vi "DAT Example.vi"() -> ()   [LabVIEW 2019]
uses:
  LV-Data/Typedefs/File Type--enum.ctl
  LV-Data/Typedefs/Dictionary--cluster.ctl
  LV-Data/LV-Data.lvclass
panel:
  out "data rows saved":i32
  in  "stop":bool
  in  "number4":dbl=7.0
  in  "number3":dbl=5.0
  in  "number2":dbl=3.0
  in  "number1":dbl
  in  "wavenames (.Vx, etc)":string[](array[string])=["time", "temp", "Bfield", "X0", "Y0", "X1", "Y1", "X2", "Y2", "X3", "Y3", "X4", "Y4", "X5", "Y5"]
  out "plot2":cluster{"X":dbl[], "Y":dbl[]}[](graph)
  out "plot1":cluster{"X":dbl[], "Y":dbl[]}[](graph)
  out "plot0":cluster{"X":dbl[], "Y":dbl[]}[](graph)
  in  "Notes":string="date and time are AUTOMATICALLY saved!\nwrite your experiment notes here"
  in  "path":path=path "C:/"
  in  "filename":string="datatest"
  # "- set path to folder\n- set base filename\n   (up to 999,999 files with same base name \n    an be written in one folder)\n- type some comments"
  # "you usually display your data as a XY\ngraphs or charts:"
  # "give everything you are saving a name,\nor else you will become confused!"
  # "initialize your file using the structure shown at right\n----------------->"
  # "wire the path using the output from the initialize step\n\ncombine all of your data using \"build  array\" function\n\nEach entry represents one data point at a partiular time"
  # "numbers can be\n saved too:"
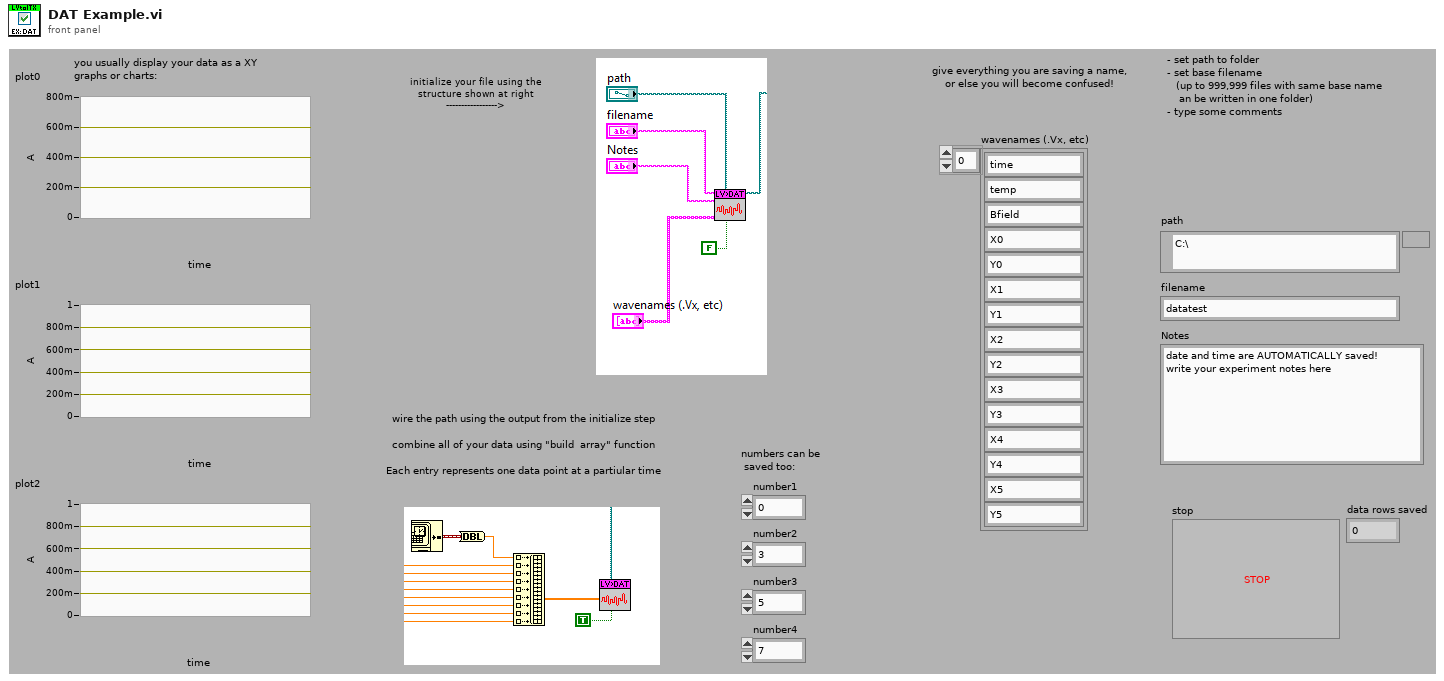
[diagram p1: front panel]
types:
  T1 = typedef "LV-Data.lvclass/Dictionary--cluster.ctl" = cluster{"key":string, "value":variant}
  T2 = typedef "LV-Data.lvclass/File Type--enum.ctl" = enum16{"DAT", "ITX", "TDMS", "VI"}
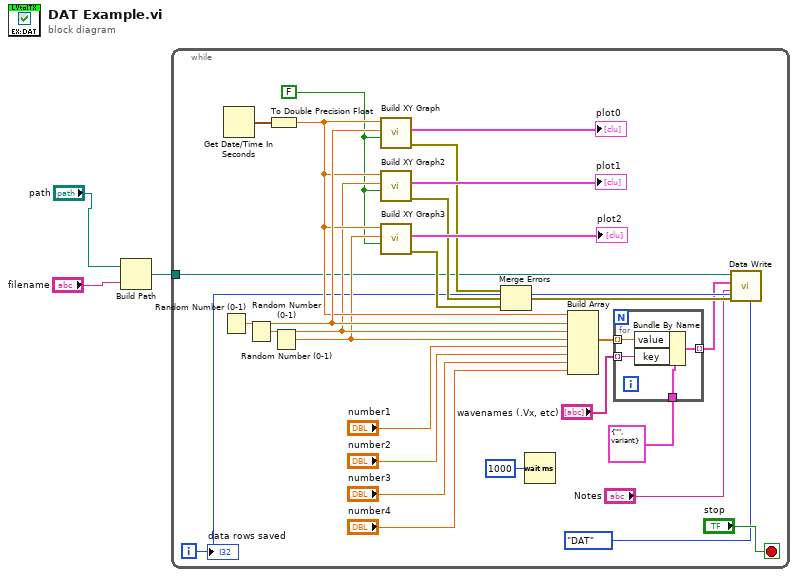
[diagram p0: block diagram]
diagram:
  n1 = Build Path(base path="path", name or relative path="filename") -> (appended path=w1:path)
  n2 = while {
    tunnel: w1 -> [w15]
    i -> [w13]
    stop <- "stop" stop-if-true
    w21 = FALSE ("Reset")
    n3 = Random Number (0-1)() -> (number: 0 to 1=w28:dbl)
    n4 = Get Date/Time In Seconds() -> (seconds since 1Jan1904=w29:timestamp)
    n5 = Random Number (0-1)() -> (number: 0 to 1=w26:dbl)
    n6 = To Double Precision Float(number=w29) -> (double precision float=w27:dbl)
    n7 = Random Number (0-1)() -> (number: 0 to 1=w25:dbl)
    n8 = call "Build XY Graph"("Reset"=w21, "Y Input"=w28, "X Input"=w27) -> ("error out"=w18:errorcluster, "XY Graph"=→"plot0":cluster{"X":dbl[], "Y":dbl[]}[])  [unwired: 7 in]
    n9 = call "Build XY Graph2"("Reset"=w21, "Y Input"=w26, "X Input"=w27) -> ("error out"=w17:errorcluster, "XY Graph"=→"plot1":cluster{"X":dbl[], "Y":dbl[]}[])  [unwired: 7 in]
    n10 = call "Build XY Graph3"("Reset"=w21, "Y Input"=w25, "X Input"=w27) -> ("error out"=w16:errorcluster, "XY Graph"=→"plot2":cluster{"X":dbl[], "Y":dbl[]}[])  [unwired: 7 in]
    n11 = Merge Errors(w18, w17, w16) -> (w14:errorcluster)
    n12 = Wait (ms)(milliseconds to wait=u32 1000) -> ()  [unwired: 1 out]
    n13 = Build Array(w27, w28, w26, w25, "number1", "number2", "number3", "number4") -> (w10:dbl[])
    n14 = for {
      tunnel: T1 {"key"="", "value"=variant} ("key-value") -> [w34]
      tunnel: w10 -> [w33] mode=indexing
      tunnel: "wavenames (.Vx, etc)" -> [w32] mode=indexing
      tunnel: [w31] -> w8 mode=indexing
      n15 = Bundle By Name(cluster=w34, "value"=w33, "key"=w32) -> (w31:T1)
    }
    n16 = call "Data Write.vi"("File Type"=File_Type--enum."DAT", "Append Index"=w13, "error in (no error)"=w14, "Notes"="Notes", "Data (Dictionary)"=w8, "path"=w15) -> ()  [unwired: 4 in, 2 out]
    "data rows saved" <- w13
  }
